vi "MW_ON.vi"() -> ()   [LabVIEW 2025]
uses:
  MW_resource_name.vi
panel:
  out "instrument handle":refnum<k15>
  out "error out 2":errorcluster {"code" format="%.0x"}
  in  "stop":bool
  out "error out":errorcluster {"code" format="%.0x"}
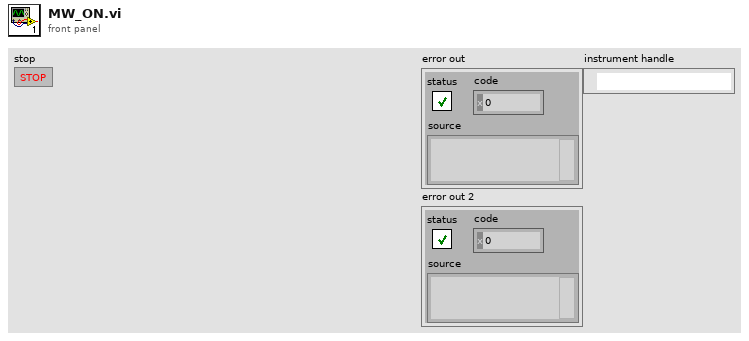
[diagram p1: front panel]
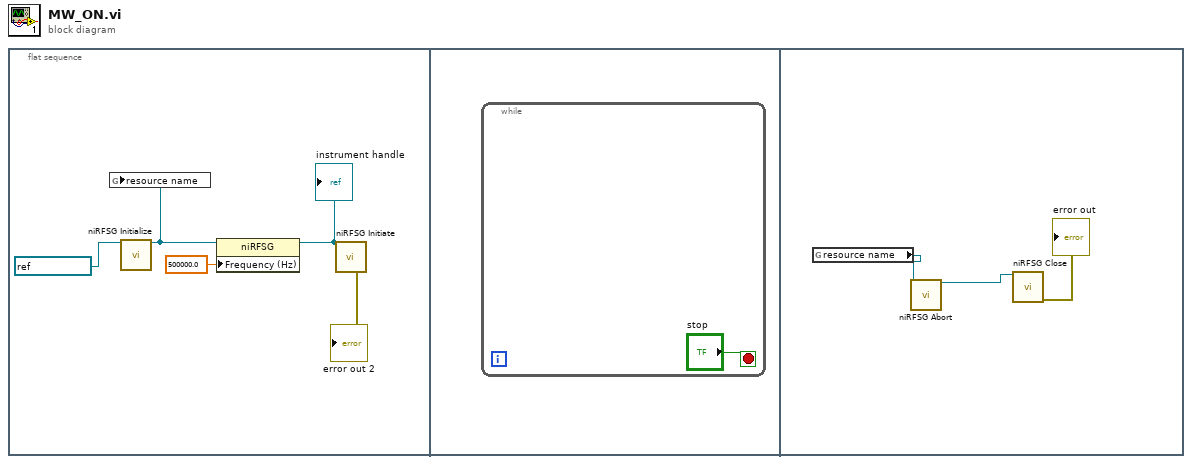
[diagram p0: block diagram]
diagram:
  n1 = flat-sequence {
    frame #0 {
      n2 = call <instrlib>:"niRFSG Initialize.vi"("resource name"=refnum<k15> "PXI1Slot2" ("instrument handle")) -> ("instrument handle"=w4:refnum<k15>)  [unwired: 13 in, 1 out]
      n3 = global write "MW_resource_name.vi" "resource name"(w4) -> ()
      n4 = property class="niRFSG"(reference=w4, "Frequency (Hz)"=500000.0 ("RF:Frequency (Hz)")) -> (reference out=w5:refnum<k15>)  [unwired: 1 in, 1 out]
      "instrument handle" <- w5
      n5 = call <instrlib>:"niRFSG Initiate.vi"("instrument handle"=w5) -> ("error out"=→"error out 2":errorcluster)  [unwired: 13 in, 1 out]
    }
    frame #1 {
      n6 = while {
        stop <- "stop" stop-if-true
      }
    }
    frame #2 {
      n7 = global read "MW_resource_name.vi" "resource name"() -> (w7:refnum<k15>)
      n8 = call <instrlib>:"niRFSG Abort.vi"("instrument handle"=w7) -> ("instrument handle out"=w8:refnum<k15>)  [unwired: 13 in, 1 out]
      n9 = call <instrlib>:"niRFSG Close.vi"("instrument handle"=w8) -> ("error out"=→"error out":errorcluster)  [unwired: 14 in]
    }
  }
